vi "Host_CommStep.vi"(4 "Transport":enum16{"TCP", "COM"}(ring), 5 "Host":string, 6 "Port":u16, 7 "COM Port":refnum<visa-resource-name>, 8 "Queue":refnum<queue>, 9 "Beat":u16, 10 "Connected":bool, 11 "PLC Conn":refnum<visa-resource-name>) -> (1 "Words":u16[](array[numeric]), 2 "Connected out":bool, 3 "PLC Conn out":refnum<visa-resource-name>)   [LabVIEW 2018]
doc: "Use this template to build a VI to use as a subVI."
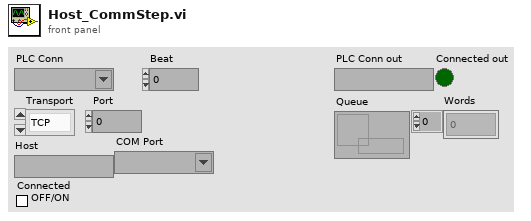
[diagram p1: front panel]
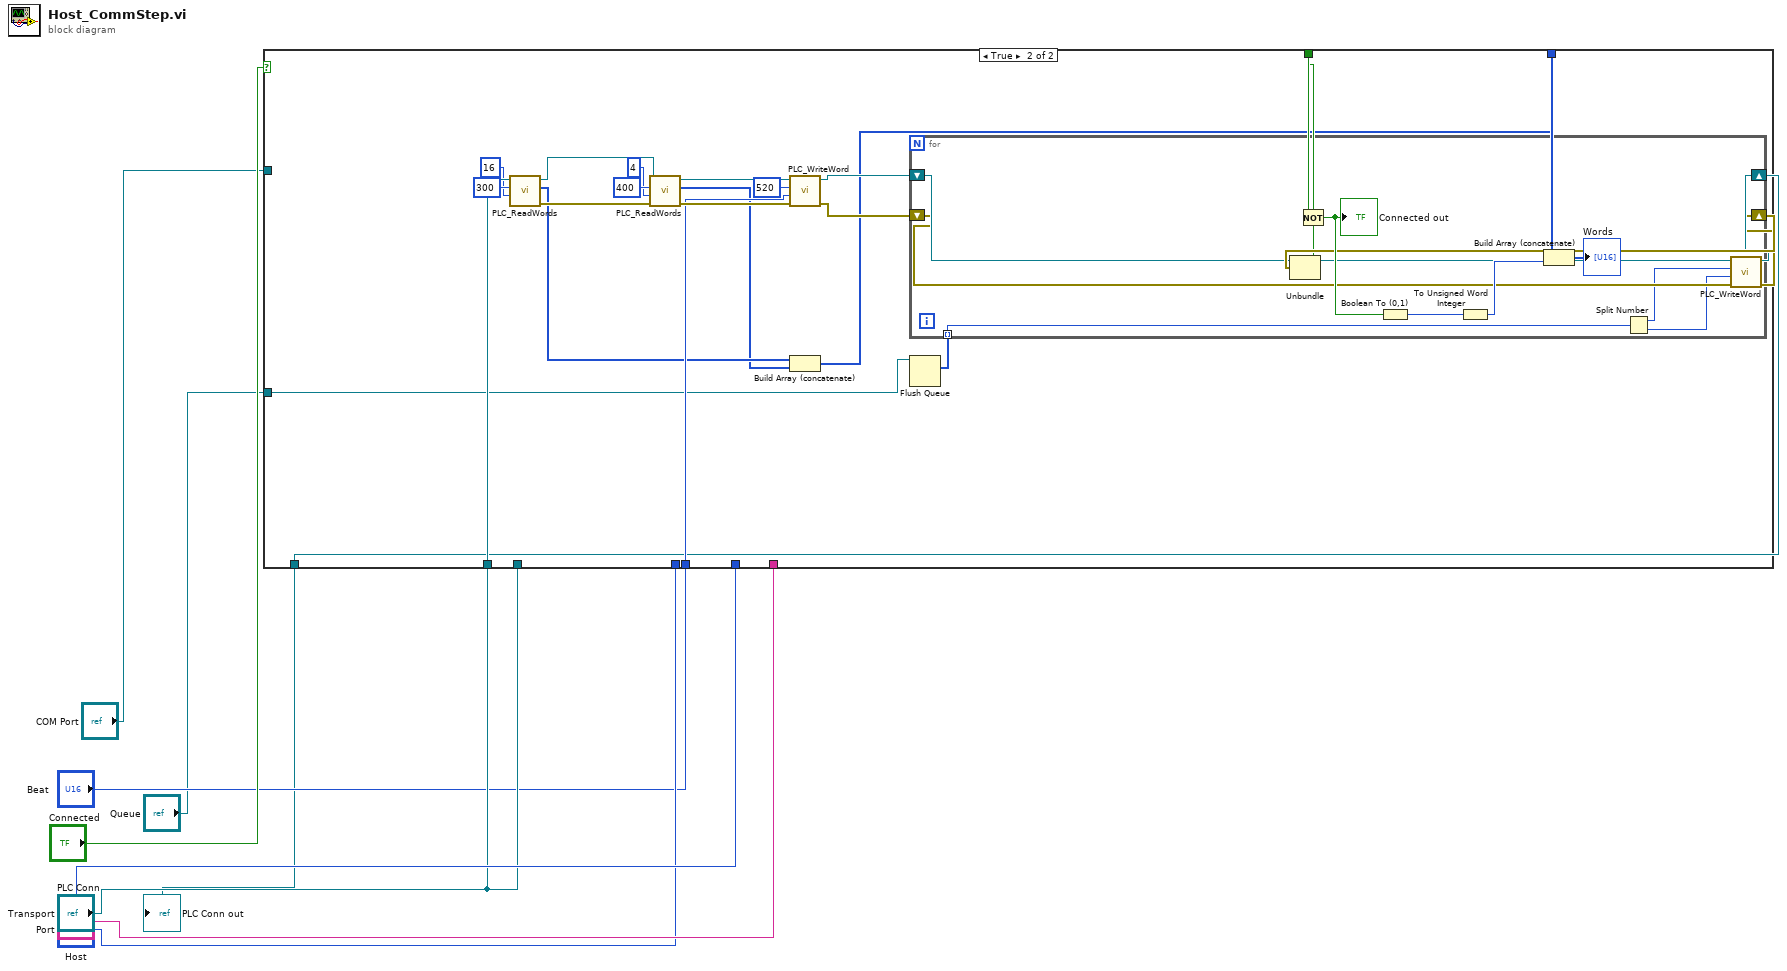
[diagram p0: block diagram]
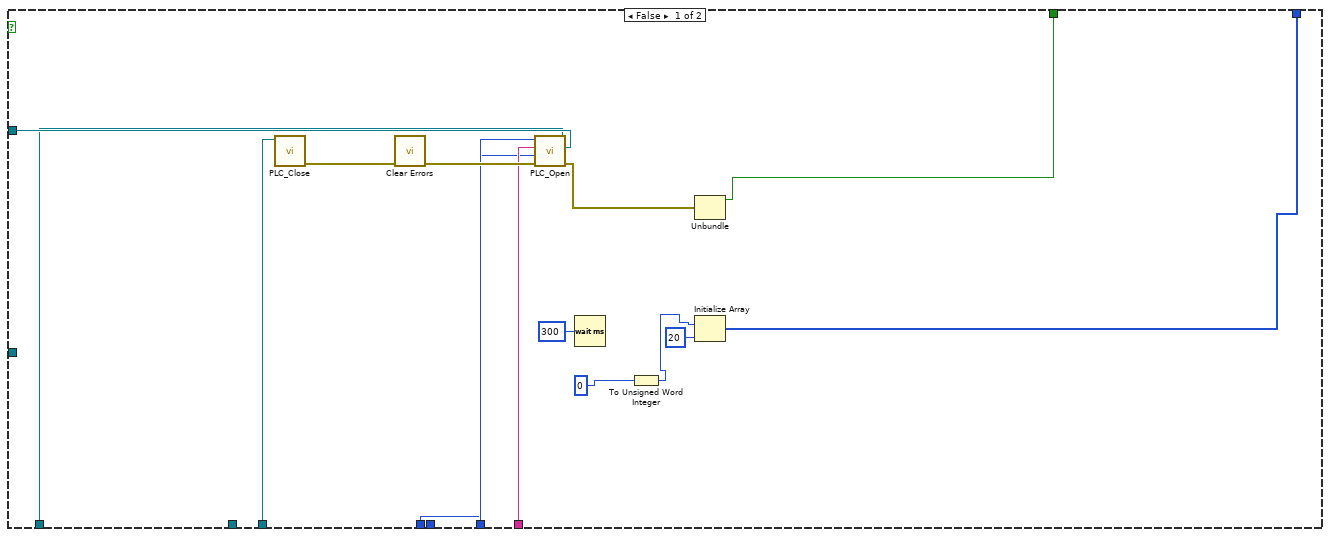
[diagram p2: hidden frame]
diagram:
  n1 = case shown="True" "Connected" {
    tunnel: "PLC Conn" -> [w30 _]
    tunnel: "Transport" -> [w27 _]
    tunnel: "Host" -> [w26 _]
    tunnel: "Port" -> [w25 _]
    tunnel: "COM Port" -> [w24 _]
    tunnel: "PLC Conn" -> [_ w51]
    tunnel: "Beat" -> [_ w41]
    tunnel: "Queue" -> [_ w38]
    tunnel: [w18 w33] -> w7
    tunnel: [w17 w32] -> w6
    tunnel: [w16 w31] -> w3
    frame False {
      n2 = call "PLC_Close.vi"("PLC Conn"=w30) -> ("error out"=w29:errorcluster)  [unwired: 10 in]
      n3 = call <vilib>:"Clear Errors.vi"("error in (no error)"=w29) -> ("error out"=w28:errorcluster)  [unwired: 5 in, 1 out]
      n4 = call "PLC_Open.vi"("COM Port"=w24, "error in (no error)"=w28, "Port"=w25, "Host"=w26, "Transport"=w27) -> ("error out"=w23:errorcluster, "PLC Conn"=w17:refnum<visa-resource-name>)  [unwired: 5 in]
      n5 = Wait (ms)(milliseconds to wait=u32 300) -> ()  [unwired: 1 out]
      n6 = To Unsigned Word Integer(number=0) -> (unsigned 16bit integer=w19:u16)
      n7 = Unbundle(w23) -> ("status"=w18:bool)  [unwired: 2 out]
      n8 = Initialize Array(w19, 20 ("dimension size")) -> (w16:u16[])
    }
    frame True {
      n9 = call "PLC_ReadWords.vi"("Count"=u16 16, "Start D"=u16 300, "PLC Conn"=w51) -> ("error out"=w45:errorcluster, "Words"=w40:u16[], "PLC Conn out"=w46:refnum<visa-resource-name>)  [unwired: 6 in]
      n10 = call "PLC_ReadWords.vi"("error in (no error)"=w45, "Count"=u16 4, "Start D"=u16 400, "PLC Conn"=w46) -> ("error out"=w43:errorcluster, "Words"=w39:u16[], "PLC Conn out"=w44:refnum<visa-resource-name>)  [unwired: 5 in]
      n11 = call "PLC_WriteWord.vi"("error in (no error)"=w43, "Value"=w41, "Address D"=u16 520, "PLC Conn"=w44) -> ("error out"=w36:errorcluster, "PLC Conn out"=w37:refnum<visa-resource-name>)  [unwired: 6 in]
      n12 = Build Array (concatenate)(w40, w39) -> (w31:u16[])
      n13 = Flush Queue(queue=w38) -> (remaining elements=w35:u32[])  [unwired: 1 in, 2 out]
      n14 = for {
        shift-right: [w53] -> w32
        shift-left: w37 -> [w57]
        shift-right: [w52] -> w34
        shift-left: w36 -> [w56]
        tunnel: w35 -> [w58] mode=indexing
        n15 = Split Number(x=w58) -> (hi(x)=w55:u16, lo(x)=w54:u16)
        n16 = call "PLC_WriteWord.vi"("error in (no error)"=w56, "Value"=w54, "Address D"=w55, "PLC Conn"=w57) -> ("error out"=w52:errorcluster, "PLC Conn out"=w53:refnum<visa-resource-name>)  [unwired: 6 in]
      }
      n17 = Unbundle(w34) -> ("status"=w33:bool)  [unwired: 2 out]
    }
  }
  "PLC Conn out" <- w6
  n18 = Not(x=w7) -> (.not. x?=w5:bool)
  "Connected out" <- w5
  n19 = Boolean To (0,1)(Boolean=w5) -> (0, 1=w4:i16)
  n20 = To Unsigned Word Integer(number=w4) -> (unsigned 16bit integer=w2:u16)
  n21 = Build Array (concatenate)(w3, w2) -> (→"Words":u16[])
